vi "OwnCompat20261012_Native_GetObjectInfo.vi"() -> ()   [LabVIEW 2024]
uses:
  <vilib>/Utility/miscctls.llb/LVBoundsTypeDef.ctl
panel:
  out "error out":errorcluster caption="错误输出"
  out "bounds":T1 caption="边界"
  out "class_name":string
  in  "object_id":u32
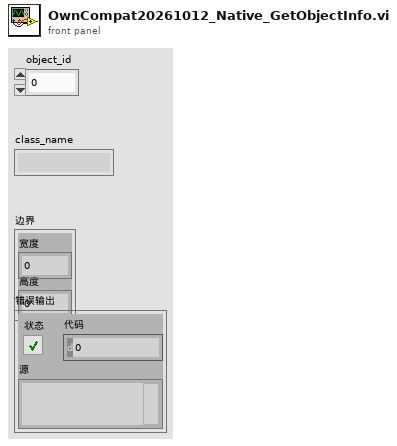
[diagram p1: front panel]
types:
  T1 = typedef "LVBoundsTypeDef.ctl" = cluster{"Width":u32, "Height":u32}
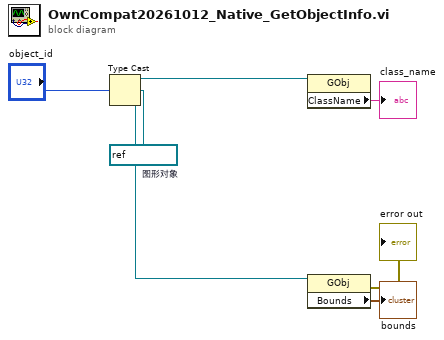
[diagram p0: block diagram]
diagram:
  w5 = refnum<vi> refnum  # 图形对象
  n1 = Type Cast ("强制类型转换")(type=w5, x="object_id") -> (*(type *) &x=w4:refnum<vi>)
  n2 = property on="属性节点" class="GObj"(reference=w4) -> ("ClassName"=→"class_name":string)  [unwired: 1 in, 2 out]
  n3 = property on="属性节点" class="GObj"(reference=w4) -> (error out=→"error out":errorcluster, "Bounds"=→"bounds":T1)  [unwired: 1 in, 1 out]
